vi "Send Message.vi"(8 "error in (no error)":errorcluster, 10 "String in":string, 11 "TCP Writer in":refnum<class "TCP Writer.lvclass">) -> (0 "error out":errorcluster, 3 "TCP Writer out":refnum<class "TCP Writer.lvclass">)   [LabVIEW 2020, in "TALOS.lvlib" / "TCP Writer.lvlib" / "TCP Writer.lvclass"]
uses:
  TCP Writer.lvclass
  C:/Users/marco/Documents/GitHub_Lab/TALOS/talos/Father of all uServices/Father of all uServices/Father of all uServices.lvclass
  TCP Writer.lvclass/TCP Writer.ctl
  Father of all uServices/Father of all uServices/Father of all uServices.lvclass/Father of all uServices.ctl
  Ancestor/Ancestor/Ancestor.lvclass/Ancestor.ctl
  TCP Writer Consumer Case Selector.ctl
  Father of all uServices/Father of all uServices Messages/Consumer Msg/Consumer Msg.lvclass/Consumer Msg.ctl
  Father of all uServices/Father of all uServices/Children Methods/Update GUI.vi
  FGV/Error Memory/Get Error Description.vi
  Support VIs/Get PC name.vi
  Ancestor/Ancestor/Read ID.vi
  Support VIs/Get Class Name.vi
  Father of all uServices/Father of all uServices Messages/Consumer Msg/Send Consumer.vi
  FGV/Error Memory/Error Memory Core.vi
  <vilib>/AdvancedString/Delimited String to 1D String Array.vi
  Support VIs/Circus Root Path.vi
  FGV/Error Memory/Error Crt Lvl checker.vi
  FGV/Error Memory/Error Memory Core.vi/40c8088d-b597-4017-91af-faa98e00292e.vi
  FGV/Error Memory/Error Memory Core.vi/d4a3ab98-063c-4e44-b43d-fbdcfe6c2be2.vi
  Father of all uServices/Father of all uServices/Father of all uServices.lvclass
  C:/Users/marco/Documents/GitHub_Lab/TALOS/builds/Actor Framework PPL/Actor Framework.lvlibp/1abvi3w/vi.lib/ActorFramework/Actor/Actor.lvclass
  Support VIs/Global Constants.vi
  Father of all uServices/Father of all uServices/Children Methods/Get GUI Item Value - String.vi
  Father of all uServices/Father of all uServices/Multiline string updater.vi
  Support VIs/Global Memory.vi
  <vilib>/Utility/LVClass/Get LV Class Name.vi
  Support VIs/Is in Packed Library.vi
  Support VIs/TALOS Root path.vi
  Support VIs/Read CSV worksheet.vi
  <vilib>/Utility/error.llb/General Error Handler.vi
  Support VIs/Error Log.vi
  builds/Actor Framework PPL/Actor Framework.lvlibp/1abvi3w/vi.lib/ActorFramework/Actor/Read Self Enqueuer.vi
  <userlib>/_OpenG.lib/lvdata/lvdata.llb/Get Strings from Enum__ogtk.vi
  builds/Actor Framework PPL/Actor Framework.lvlibp/1abvi3w/vi.lib/ActorFramework/Message Enqueuer/Enqueue.vi
  Ancestor/Ancestor/Ancestor.lvclass
  <vilib>/Comparison/Equal/Equal Functor/Equal Functor.lvclass
  Father of all uServices/Father of all uServices Messages/Consumer Msg/Consumer Msg.lvclass
  TALOS.lvlib
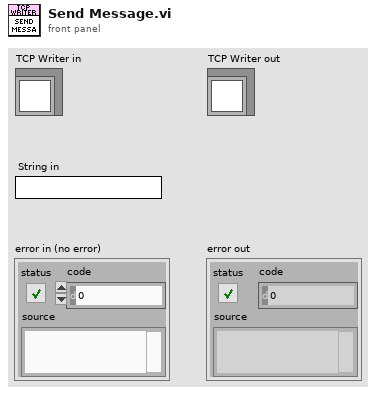
[diagram p1: front panel]
types:
  T1 = typedef "TALOS.lvlib/TCP Writer.lvlib/TCP Writer.lvclass/TCP Writer Consumer Case Selector.ctl" = enum16{"Send message", "Idle", "Check Connection", "Open connection", "Set Client ID"}
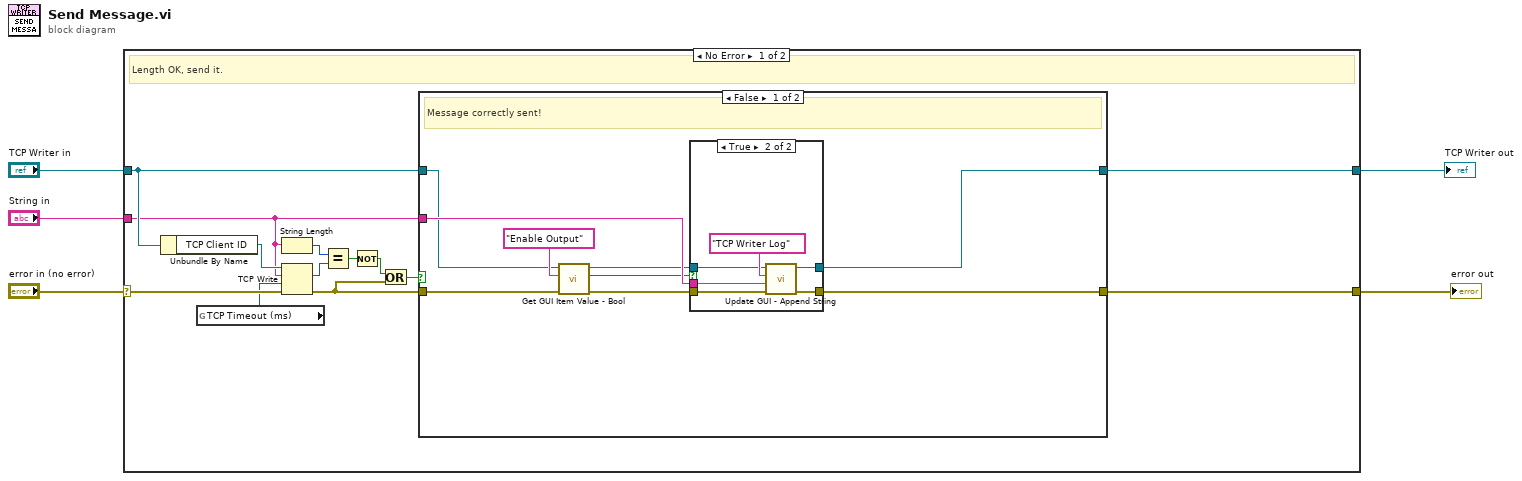
[diagram p0: block diagram]
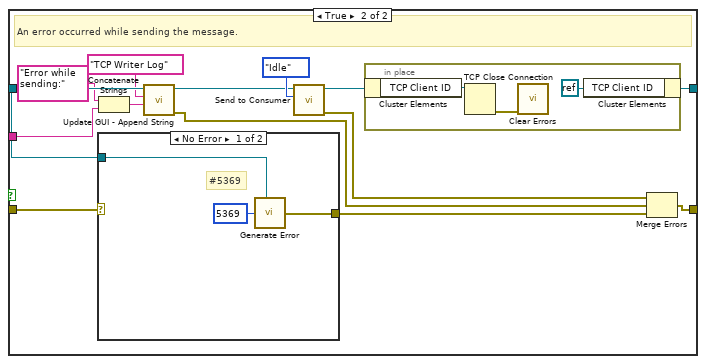
[diagram p3: hidden frame]
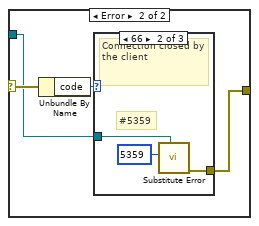
[diagram p4: hidden frame]
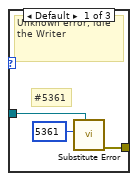
[diagram p5: hidden frame]
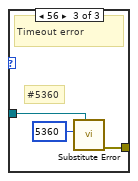
[diagram p6: hidden frame]
diagram:
  n1 = case shown="No Error" "error in (no error)" {
    selector: "error in (no error)" -> [w16 w70]
    tunnel: [w18 w70] -> w1
    tunnel: "TCP Writer in" -> [w15 w69]
    tunnel: "String in" -> [w6 _]
    tunnel: [w17 w69] -> w2
    frame No Error {
      # "Length OK, send it."
      n2 = Unbundle By Name(w15) -> ("TCP Client ID"=w14:refnum<k5>)
      n3 = global read "Global Constants.vi" "TCP Timeout (ms)"() -> (w13:i32)
      n4 = String Length(string=w6) -> (length=w12:i32)
      n5 = TCP Write(connection ID=w14, data in=w6, error in (no error)=w16, 9:w13) -> (bytes written=w11:i32, error out=w7:errorcluster)  [unwired: 1 out]
      n6 = Equal?(x=w12, y=w11) -> (x = y?=w10:bool)
      n7 = Not(x=w10) -> (.not. x?=w8:bool)
      n8 = Or(x=w8, y=w7) -> (x .or. y?=w9:bool)
      n9 = case shown="False" w9 {
        tunnel: w15 -> [w20 w49]
        tunnel: [w25 w46] -> w18
        tunnel: [w27 w36] -> w17
        tunnel: w7 -> [w23 w44]
        tunnel: w6 -> [w26 w39]
        frame False {
          # "Message correctly sent!"
          n10 = call "Get GUI Item Value - Bool.vi"("error in (no error)"=w23, "FP Item Name"="Enable Output" ("Parameter Name"), "uService Template in"=w20) -> ("error out"=w22:errorcluster, "Value"=w21:bool, "uService Template out"=w19:refnum<class "TCP Writer.lvclass">)  [unwired: 6 in]
          n11 = case shown="True" w21 {
            tunnel: w22 -> [w29 w35]
            tunnel: [w29 w34] -> w25
            tunnel: w26 -> [_ w33]
            tunnel: [w28 w31] -> w27
            tunnel: w19 -> [w28 w30]
            frame False {
            }
            frame True {
              n12 = call "Update GUI - Append String.vi"("error in (no error)"=w35, "String"=w33, "GUI Item Name"="TCP Writer Log", "Father of all uServices in"=w30) -> ("error out"=w34:errorcluster, "Father of all uServices out"=w31:refnum<class "TCP Writer.lvclass">)  [unwired: 6 in]
            }
          }
        }
        frame True {
          # "An error occurred while sending the message."
          n13 = case shown="No Error" w44 {
            selector: w44 -> [_ w54]
            tunnel: [w52 w55] -> w45
            tunnel: w49 -> [w51 w53]
            frame No Error {
              # "#5369"
              n14 = call "Generate Error.vi"("Class"=w51, "Error Code"=5369) -> ("error out"=w52:errorcluster)  [unwired: 5 in]
            }
            frame Error {
              n15 = Unbundle By Name(w54) -> ("code"=w56:i32)
              n16 = case shown="66" w56 {
                tunnel: [w58 w62 w64] -> w55
                tunnel: w53 -> [w57 w60 w63]
                frame Default {
                  # "#5361"
                  # "Unknown error, idle the Writer"
                  n17 = call "Substitute Error.vi"("LabVIEW Object"=w57, "Error Code"=5361) -> ("error out"=w58:errorcluster)  [unwired: 9 in]
                }
                frame 66 {
                  # "#5359"
                  # "Connection closed by the client"
                  n18 = call "Substitute Error.vi"("LabVIEW Object"=w60, "Error Code"=5359) -> ("error out"=w62:errorcluster)  [unwired: 9 in]
                }
                frame 56 {
                  # "#5360"
                  # "Timeout error"
                  n19 = call "Substitute Error.vi"("LabVIEW Object"=w63, "Error Code"=5360) -> ("error out"=w64:errorcluster)  [unwired: 9 in]
                }
              }
            }
          }
          n20 = Concatenate Strings("Error while sending:" ("GUI Item Name"), w39) -> (w38:string)
          n21 = call "Update GUI - Append String.vi"("String"=w38, "GUI Item Name"="TCP Writer Log", "Father of all uServices in"=w49) -> ("error out"=w41:errorcluster, "Father of all uServices out"=w42:refnum<class "TCP Writer.lvclass">)  [unwired: 7 in]
          n22 = call "Send to Consumer.vi"("Case ID"=TCP_Writer_Consumer_Case_Selector."Idle" ("TCP Listener Consumer Case Selector"), "uService Template in"=w42) -> ("error out"=w48:errorcluster, "uService Template out"=w37:refnum<class "TCP Writer.lvclass">)  [unwired: 8 in]
          n23 = in-place {
            n24 = in-place-cluster #1(w37) -> ("TCP Client ID"=w68:refnum<k5>)
            n25 = TCP Close Connection(connection ID=w68) -> (error out=w67:errorcluster)  [unwired: 2 in, 1 out]
            n26 = call <vilib>:"Clear Errors.vi"("error in (no error)"=w67) -> ()  [unwired: 5 in, 2 out]
            n27 = in-place-cluster #1("TCP Client ID"=refnum<k0> refnum) -> (w36:refnum<class "TCP Writer.lvclass">)
          }
          n28 = Merge Errors(w48, w41, w45) -> (w46:errorcluster)
        }
      }
    }
    frame Error {
      # "DO not kill the connection: something went wrong with the part generating the message, not the TCP connection itself."
      # "Something went wrong: just let the error go out."
    }
  }
  "TCP Writer out" <- w2
  "error out" <- w1
